vi "Alarms.CacheCurrentValues.vi"(7 "Station.ID":string, 8 "error in (no error)":errorcluster, 11 "ListBox in":refnum<vi>) -> (0 "error out":errorcluster, 3 "Alarms":T1[](array[typedef]) {"Delay" format="%.2f"; "Low Limit" format="%.2f"; "High Limit" format="%.2f"})   [LabVIEW 2015, in "Single Station Execution.lvlib"]
uses:
  Single Station Execution.lvlib
  Types/Config.AlarmSettings.ctl
  NationalInstruments.VeriStand
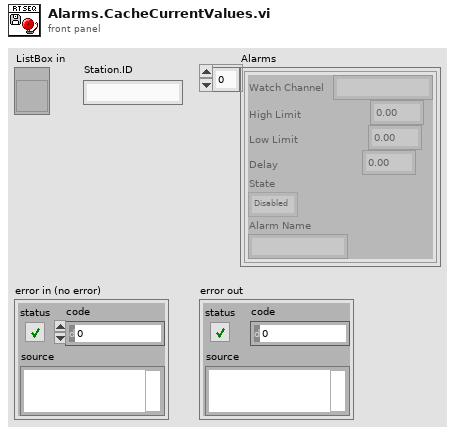
[diagram p1: front panel]
types:
  T1 = typedef "Single Station Execution.lvlib/Config.AlarmSettings.ctl" = cluster{"Watch Channel":string, "High Limit":dbl, "Low Limit":dbl, "Delay":dbl, "State":enum16{"Disabled", "Enabled", "Tripped", "Delayed Trip", "Indicate"}, "Alarm Name":string}
  T2 = enum16{"Disabled", "Enabled", "Tripped", "Delayed Trip", "Indicate"}
  T3 = typedef "NI_VS Alarm ExecutionAPI.lvlib/AlarmInfo.ctl" = cluster{"Watch Channel":string, "High Limit Constant":bool, "High Limit Channel":string, "High Limit":dbl, "Low Limit Constant":bool, "Low Limit Channel":string, "Low Limit":dbl, "Procedure Name":string, "Delay":dbl, "Trip Value":dbl, "Priority":enum16{"Low", "Medium", "High"}, "State":enum16{"Disabled", "Enabled", "Tripped", "Delayed Trip", "Indicate"}, "Mode":enum16{"Normal", "Indicate Only"}, "Group Number":u32, "Priority Number":u32, "Name":string, "Full Name":string}
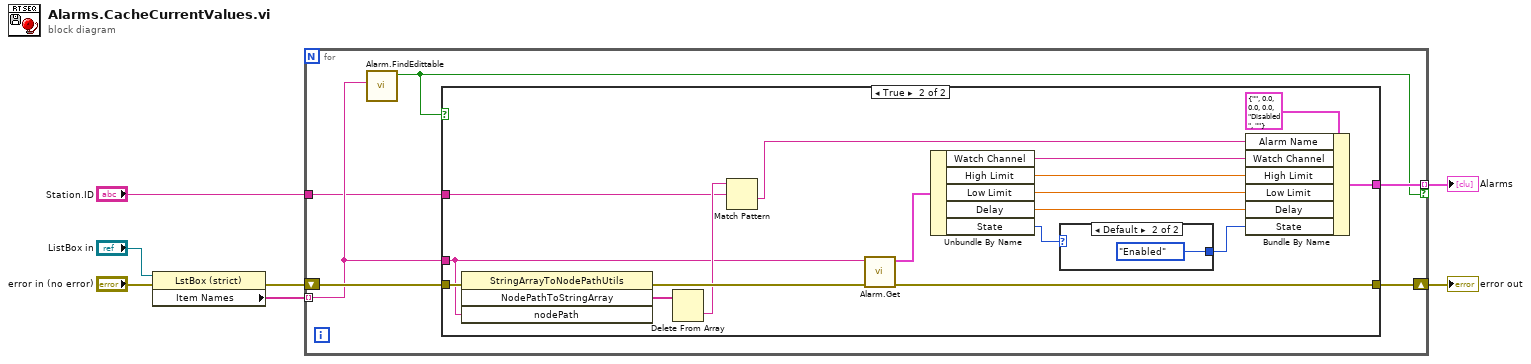
[diagram p0: block diagram]
diagram:
  n1 = property class="LstBox (strict)"(reference="ListBox in", error in="error in (no error)") -> (error out=w5:errorcluster, "Item Names"=w4:string[])  [unwired: 1 out]
  n2 = for {
    tunnel: w4 -> [w10] mode=indexing
    shift-right: [w12] -> w6
    shift-left: w5 -> [w13]
    tunnel: [w11] -> w7 mode=indexing if=w9
    tunnel: "Station.ID" -> [w8]
    n3 = call "Alarm.FindEdittable.vi"("String"=w10) -> ("Edit?"=w9:bool)  [unwired: 10 in]
    n4 = case shown="True" w9 {
      tunnel: w13 -> [w14 w21]
      tunnel: [w14 w31] -> w12
      tunnel: [_ w24] -> w11
      tunnel: w10 -> [_ w17]
      tunnel: w8 -> [_ w15]
      frame False {
      }
      frame True {
        n5 = invoke class="StringArrayToNodePathUtils" method="NodePathToStringArray"(error in=w21, "nodePath"=w17) -> (error out=w20:errorcluster, "NodePathToStringArray"=w19:string[])  [unwired: 2 in, 2 out]
        n6 = Delete From Array(array=w19) -> (deleted portion=w18:string)  [unwired: 2 in, 1 out]
        n7 = Match Pattern(string=w18, regular expression=w15) -> (after substring=w16:string)  [unwired: 1 in, 3 out]
        n8 = call "Alarm.Get.vi"("error in (no error)"=w20, "Alarm"=w17) -> ("error out"=w31:errorcluster, "Alarm Data"=w30:T3)  [unwired: 8 in]
        n9 = Unbundle By Name(w30) -> ("Watch Channel"=w28:string, "High Limit"=w27:dbl, "Low Limit"=w26:dbl, "Delay"=w25:dbl, "State"=w23:T2)
        n10 = case shown="Default" w23 {
          selector: w23 -> [w32 _]
          tunnel: [w32 T2."Enabled" ("State")] -> w22
          frame "Disabled" {
          }
          frame Default {
          }
        }
        n11 = Bundle By Name(cluster=T1 {"Watch Channel"="", "High Limit"=0.0, "Low Limit"=0.0, "Delay"=0.0, "State"=enum."Disabled", "Alarm Name"=""} ("Alarm.Settings"), "Alarm Name"=w16, "Watch Channel"=w28, "High Limit"=w27, "Low Limit"=w26, "Delay"=w25, "State"=w22) -> (w24:T1)
      }
    }
  }
  "Alarms" <- w7
  "error out" <- w6
